vi "Read Event Ref.vi"(8 "error in (no error)":errorcluster, 11 "UserEventActivationHandler in":refnum<class "UserEventActivationHandler.lvclass">) -> (0 "error out":errorcluster, 2 "Event Ref":refnum<user-event>, 3 "UserEventActivationHandler out":refnum<class "UserEventActivationHandler.lvclass">)   [LabVIEW 2026, in "ToastNotification.lvlib" / "UserEventActivationHandler.lvclass"]
doc: "Return a borrowed reference to the User Event created by Initialize. Read this property from the initialized handler returned by ToastService.Initialize, then register for this event in the calling application. The event payload contains Activation and the callback conversion error. The handler owns the event; the caller owns its event registration. Unregister the receiving registration before service Close destroys the event. Reading this property does not create an event."
uses:
  UserEventActivationHandler.lvclass
  Activation Event Data.ctl
  ToastNotification/Activation.ctl
  ToastNotification/Argument.ctl
  UserEventActivationHandler.lvclass/UserEventActivationHandler.ctl
  ToastNotification/ToastNotification.lvlib
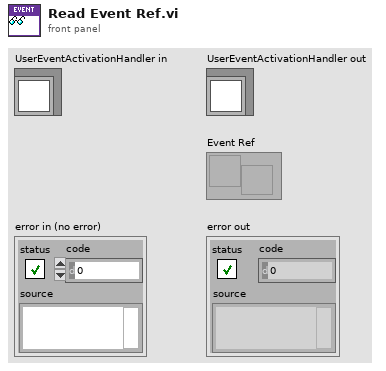
[diagram p1: front panel]
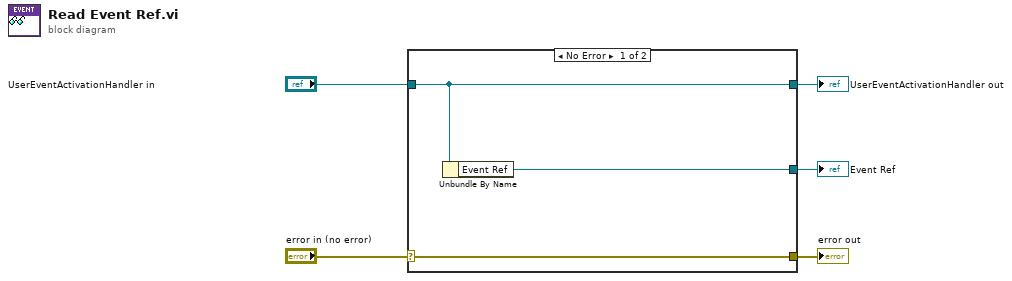
[diagram p0: block diagram]
diagram:
  n1 = case shown="No Error" "error in (no error)" {
    selector: "error in (no error)" -> [w8 w9]
    tunnel: [w8 w9] -> w4
    tunnel: [w7 w10] -> w2
    tunnel: "UserEventActivationHandler in" -> [w7 w10]
    tunnel: [w6 _] -> w1
    frame No Error {
      n2 = Unbundle By Name(w7) -> ("Event Ref"=w6:refnum<user-event>)
    }
    frame Error {
    }
  }
  "error out" <- w4
  "UserEventActivationHandler out" <- w2
  "Event Ref" <- w1
